vi "Data Adjust.vi"(10 "Data Serie":T1, 11 "Data Adjust":T2 {"偏移" format="%.2f"; "倍率" format="%.2f"}) -> (3 "Data Serie":T1)   [LabVIEW 2020, in "Data Viewer.lvlib" / "Data Viewer.lvclass"]
uses:
  Data Viewer.lvclass
  Data Adjust.ctl
  Data Action Type.ctl
  Data Serie--cluster.ctl
  Data Viewer.lvlib
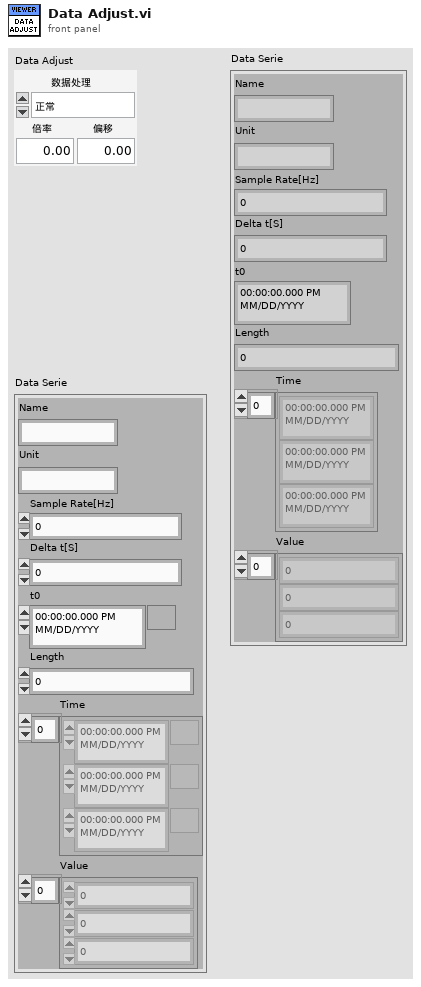
[diagram p1: front panel]
types:
  T1 = typedef "Data Viewer.lvlib/Data Serie--cluster.ctl" = cluster{"Name":string, "Unit":string, "Sample Rate[Hz]":dbl, "Delta t[S]":dbl, "t0":timestamp, "Length":i32, "Time":timestamp[], "Value":dbl[]}
  T2 = typedef "Data Viewer.lvlib/Data Viewer.lvclass/Data Adjust.ctl" = cluster{"数据处理":T3, "倍率":dbl, "偏移":dbl}
  T3 = typedef "Data Viewer.lvlib/Data Viewer.lvclass/Data Action Type.ctl" = enum16{"正常", "绝对值", "取负", "取对数"}
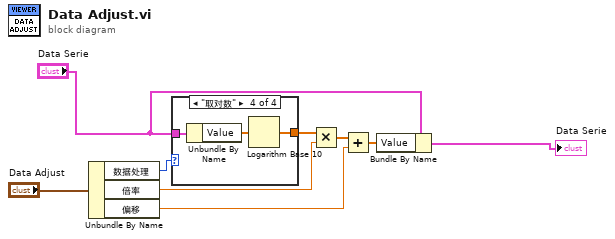
[diagram p0: block diagram]
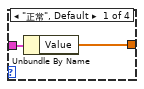
[diagram p2: hidden frame]
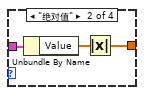
[diagram p3: hidden frame]
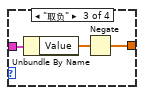
[diagram p4: hidden frame]
diagram:
  n1 = Unbundle By Name("Data Adjust") -> ("数据处理"=w4:T3, "倍率"=w6:dbl, "偏移"=w9:dbl)
  n2 = case shown="\"取对数\"" w4 {
    tunnel: "Data Serie" -> [w11 w13 w16 w20]
    tunnel: [w10 w12 w15 w18] -> w5
    frame "正常", Default {
      n3 = Unbundle By Name(w11) -> ("Value"=w10:dbl[])
    }
    frame "绝对值" {
      n4 = Unbundle By Name(w13) -> ("Value"=w14:dbl[])
      n5 = Absolute Value(x=w14) -> (abs(x)=w12:dbl[])
    }
    frame "取负" {
      n6 = Unbundle By Name(w16) -> ("Value"=w17:dbl[])
      n7 = Negate(x=w17) -> (-x=w15:dbl[])
    }
    frame "取对数" {
      n8 = Unbundle By Name(w20) -> ("Value"=w19:dbl[])
      n9 = Logarithm Base 10(1:w19) -> (0:w18:dbl[])
    }
  }
  n10 = Multiply(x=w5, y=w6) -> (x*y=w8:dbl[])
  n11 = Add(x=w8, y=w9) -> (x+y=w7:dbl[])
  n12 = Bundle By Name(cluster="Data Serie", "Value"=w7) -> (→"Data Serie":T1)
